vi "UI (The Advanced).vi"() -> ()   [LabVIEW 2017, in "UI.lvlib"]
doc: "The Queued Message Handler of a Worker."
uses:
  UI.lvlib
  _support/Analysis Window Type.ctl
  _support/UI State.ctl
  1af51285-6659-428e-9c15-de70f1a207c9.vi
  1756710f-d813-4077-a3f9-6f06171a4225.vi
  b1498353-a107-4479-98d0-7e76c0451ff6.vi
  242d01f8-d211-4c25-bb6c-8191a2acbe42.vi
  da0d510b-1f54-4e49-9d1f-893e7e8abfcf.vi
  e403ca69-710b-4b23-8527-f02bfa86df9b.vi
  <userlib>/_NEVSTOP/Communicable State Machine(CSM)/AdvanceAPI/CSM - Revert Arguments-Safe String.vi
  <userlib>/_NEVSTOP/Communicable State Machine(CSM)/_Shared/Trim Single-line Text.vi
  <userlib>/_NEVSTOP/Communicable State Machine(CSM)/AdvanceAPI/CSM - Make String Arguments Safe.vi
  <userlib>/_NEVSTOP/Communicable State Machine(CSM)/AdvanceAPI/CSM - Break Down Multiple States String.vi
  <userlib>/_NEVSTOP/Communicable State Machine(CSM)/AdvanceAPI/CSM - Keywords.vi
  <userlib>/_NEVSTOP/Communicable State Machine(CSM)/addons/INI-Static-Variable-Support/_Support/instances/_CSM - Read File Logger Configuration - v1.0.vi
  <userlib>/_NEVSTOP/Communicable State Machine(CSM)/addons/API-String-Arugments-Support/_Support/Convert API String Arguments to Data(variant).vi
  <userlib>/_NEVSTOP/Communicable State Machine(CSM)/addons/API-String-Arugments-Support/_Support/Query Data as API String Arguments(variant).vi
  <userlib>/_NEVSTOP/Communicable State Machine(CSM)/addons/MassData-Parameter/_support/FGV-MassData(lvlibp).vi
  <userlib>/_NEVSTOP/Communicable State Machine(CSM)/_Polymophic/Add State(s) to Queue By BOOL(Element).vi
  <userlib>/_NEVSTOP/Communicable State Machine(CSM)/_Polymophic/CSM - Replace Marks in Messages.vi
  Acquisition/Acquisition.lvlib
  Logging/Logging.lvlib
  <userlib>/_NEVSTOP/Communicable State Machine(CSM)/Communicable State Machine.lvlib
  <userlib>/_NEVSTOP/Communicable State Machine(CSM)/addons/MassData-Parameter/CSM MassData Parameter Support.lvlib
  <userlib>/_NEVSTOP/Communicable State Machine(CSM)/addons/INI-Static-Variable-Support/INI-Static-Variable-Support.lvlib
  Algorithm/Algorithm.lvlib
  <userlib>/_NEVSTOP/Communicable State Machine(CSM)/addons/Logger/CSM File Logger.lvlib
  <userlib>/_NEVSTOP/Communicable State Machine(CSM)/addons/Watchdog/CSM Watchdog.lvlib
  SoundInput-DAQ/SoundInput-DAQ.lvlib
  <userlib>/_NEVSTOP/Communicable State Machine(CSM)/_Polymophic/Build Synchronous Message with Arguments.vi
panel:
  in  "Data Source":enum16{"Simulated Waveform", "Sound Card"}(ring) caption="Data Source: \nSelect Before Running"
  out "WaveformGraph":waveform(dbl)[](graph)
  in  "Analysis Window 1":T1
  out "AnalysisWnd 1":cluster{"f0":dbl, "df":dbl, "magnitude":dbl[]}[](graph)
  in  "Analysis Window 2":T1
  out "AnalysisWnd 2":cluster{"f0":dbl, "df":dbl, "magnitude":dbl[]}[](graph)
  in  "Settings":bool
  in  "Start":bool
  in  "Stop":bool
  out "Status":string
  in  "Exit":bool
  # "Continuous Measurement and Data Logger - CSM Version"
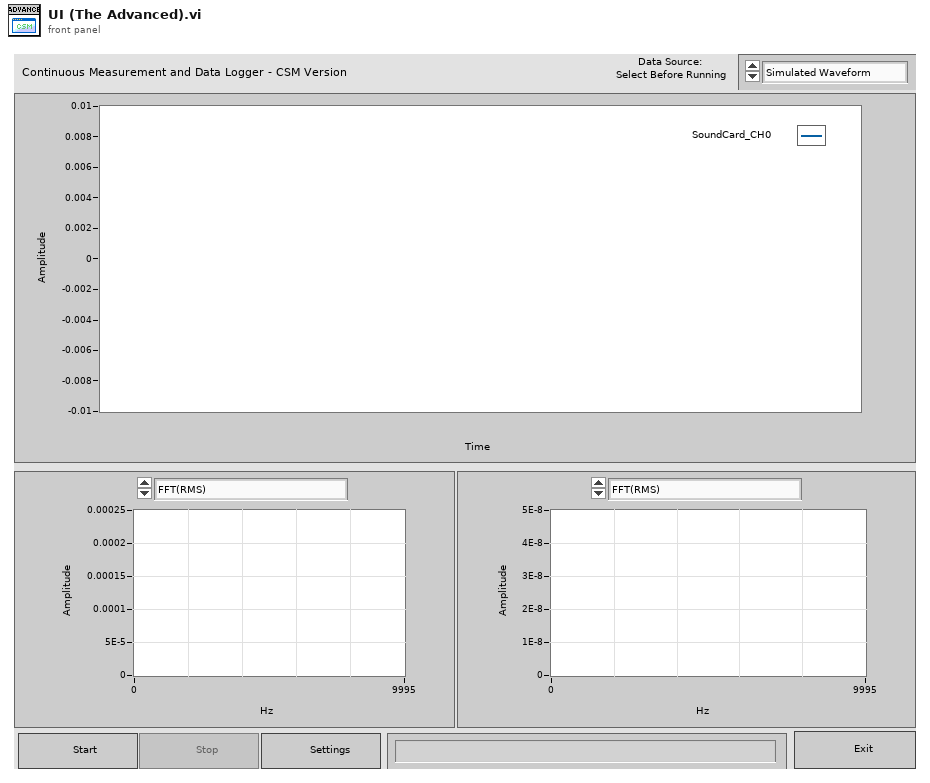
[diagram p1: front panel]
types:
  T1 = typedef "UI.lvlib/Analysis Window Type.ctl" = enum16{"FFT(RMS)", "FFT(Peak)", "Power Spectrum"}
  T2 = cluster{"Enable":bool, "Limit":cluster{"FileSize":i64, "FileNum":i32}, "Timestamp.Format":string, "AutoExit":bool}
  T3 = enum32{"Invalid", "Standard", "Closed", "Hidden", "Minimized", "Maximized"}
  T4 = enum32{"invalid app kind", "Development System", "Run Time System", "Student Edition", "Embedded LabVIEW", "Evaluation", "Custom"}
  T5 = typedef "UI.lvlib/UI State.ctl" = enum16{"Idle", "Acquiring and Logging", "Waiting for Exit", "Waiting for Exit (Acq Stopped)", "Waiting for Exit (Log Stopped)", "Waiting for Stop", "Waiting for Stop (Acq Stopped)", "Waiting for Stop (Log Stopped)"}
  T6 = enum32{"Invalid", "Default", "Floating", "Floating/Auto-Hide", "Modal"}
  T7 = typedef "Communicable State Machine.lvlib/_CSM_Response Source Message.ctl" = cluster{"‘State":string, "’Arguments":string, "’Error":errorcluster}
  T8 = cluster{"Current VI Reference":refnum<vi>, "Close Panel on Exit?":bool}
  T9 = cluster{"Core":cluster{"Current VI Reference":refnum<vi>, "Close Panel on Exit?":bool}, "UI Refs":cluster{"Start Ref":refnum<vi>, "Stop Ref":refnum<vi>, "Settings Ref":refnum<vi>, "Exit Ref":refnum<vi>, "Status Ref":refnum<vi>, "Data Ref":refnum<vi>, "Data Source Ref":refnum<vi>}, "State":T5, "Relationships":string}
  T10 = cluster{"Start Ref":refnum<vi>, "Stop Ref":refnum<vi>, "Settings Ref":refnum<vi>, "Exit Ref":refnum<vi>, "Status Ref":refnum<vi>, "Data Ref":refnum<vi>, "Data Source Ref":refnum<vi>}
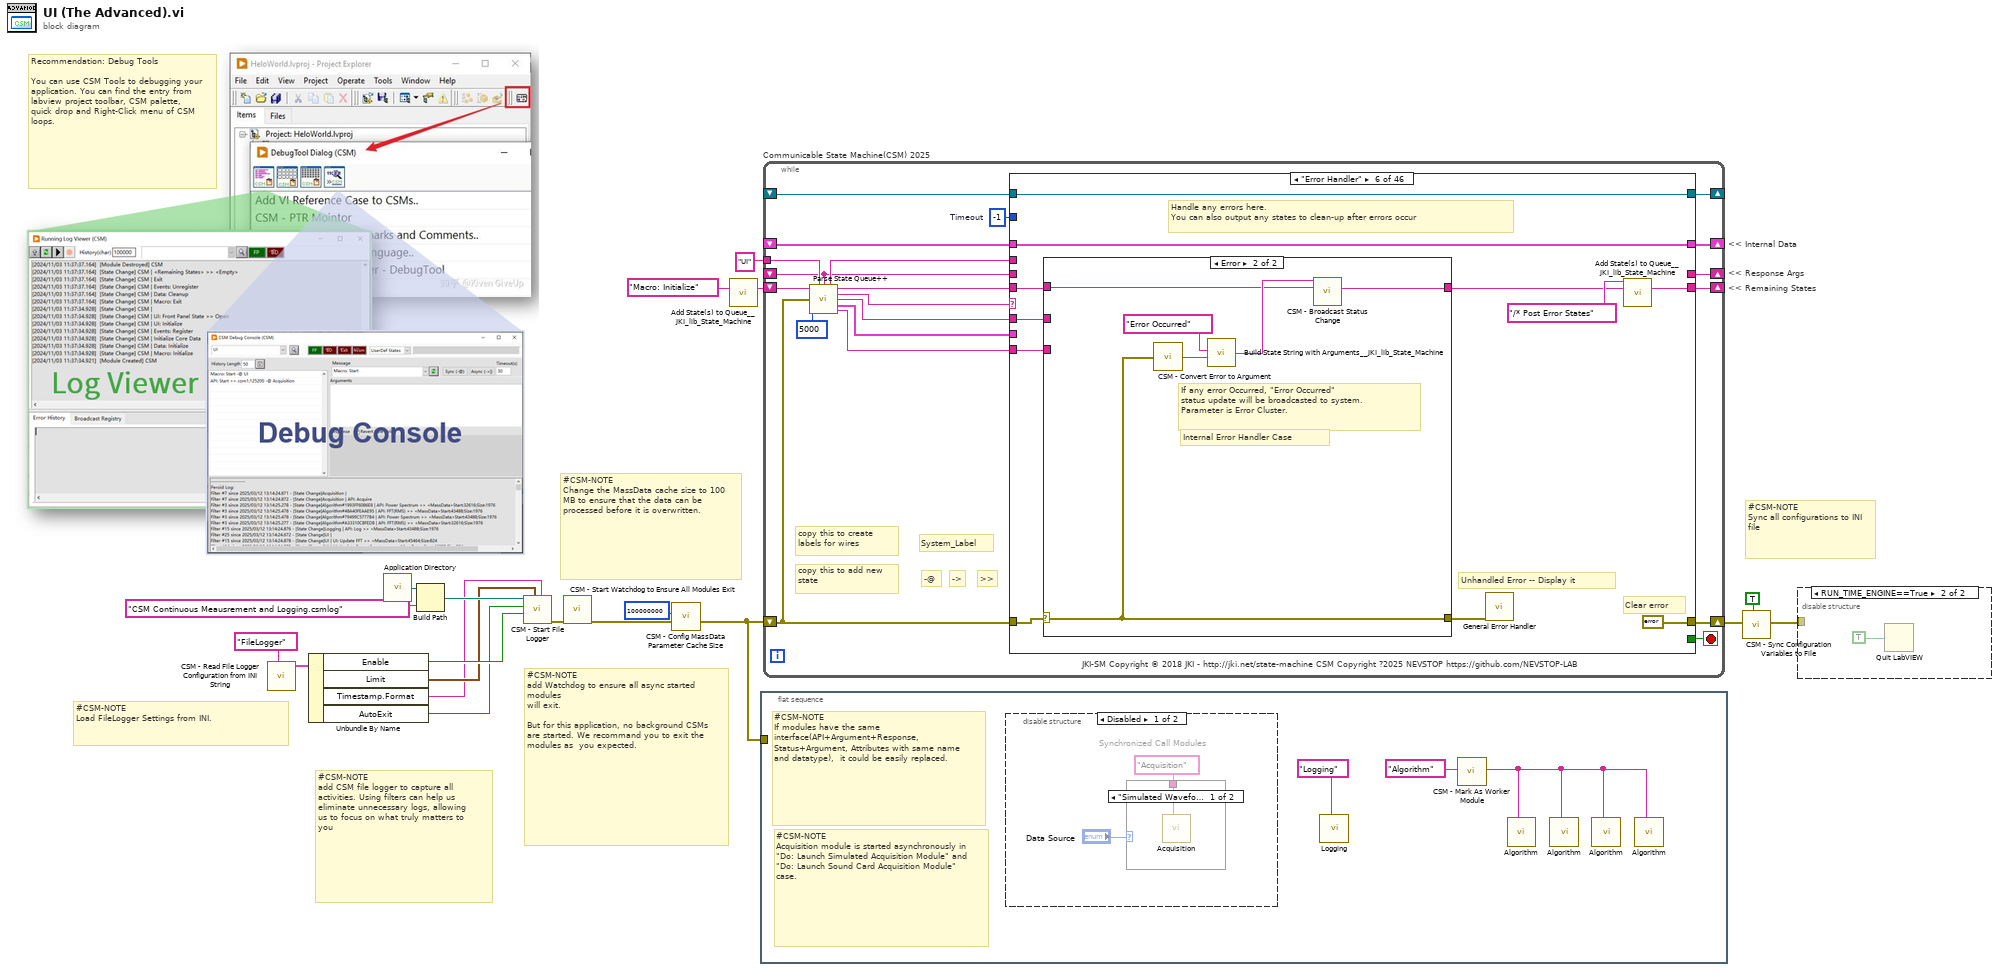
[diagram p0: block diagram]
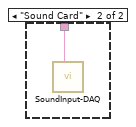
[diagram p3: hidden frame]
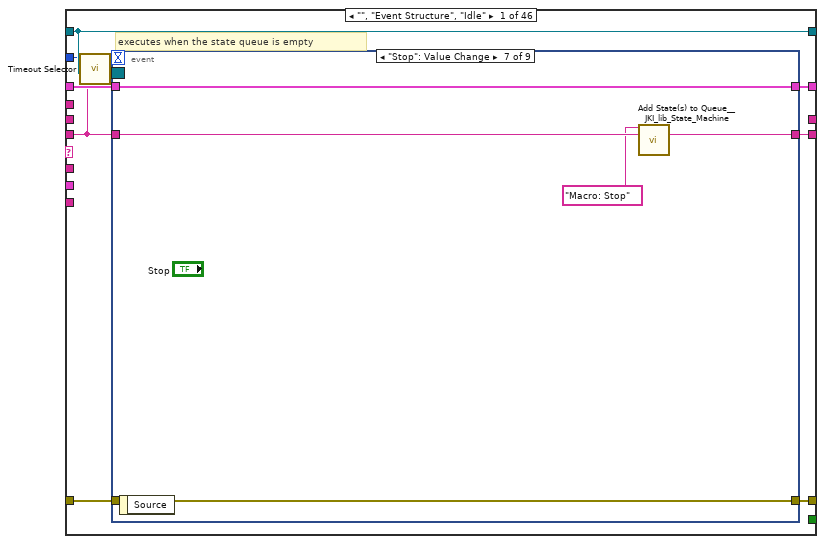
[diagram p5: hidden frame]
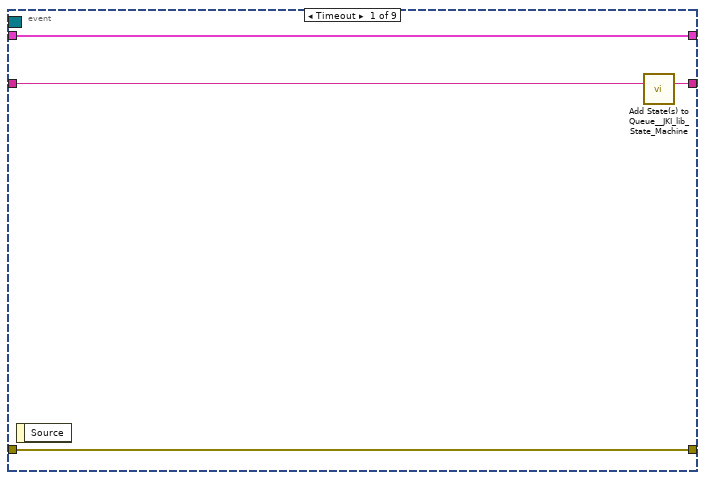
[diagram p6: hidden frame]
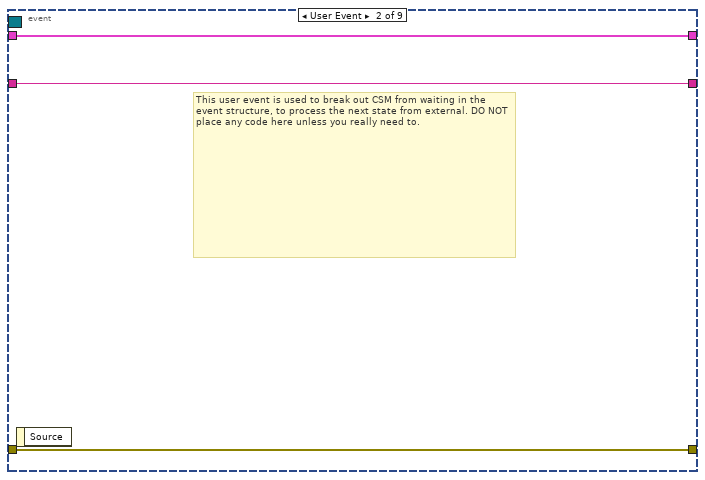
[diagram p7: hidden frame]
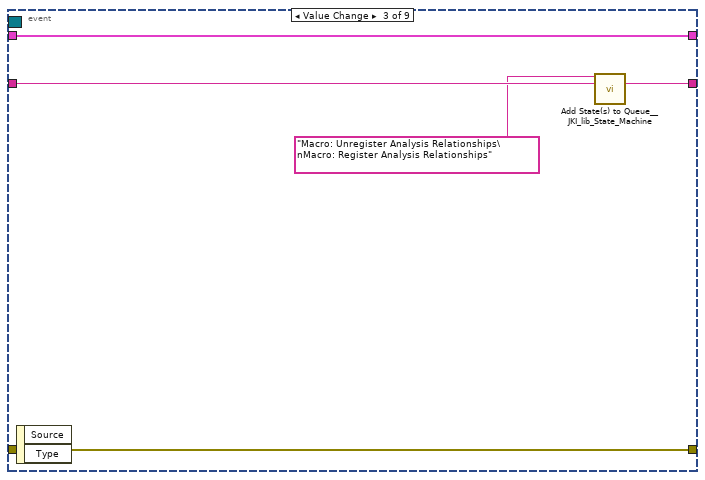
[diagram p8: hidden frame]
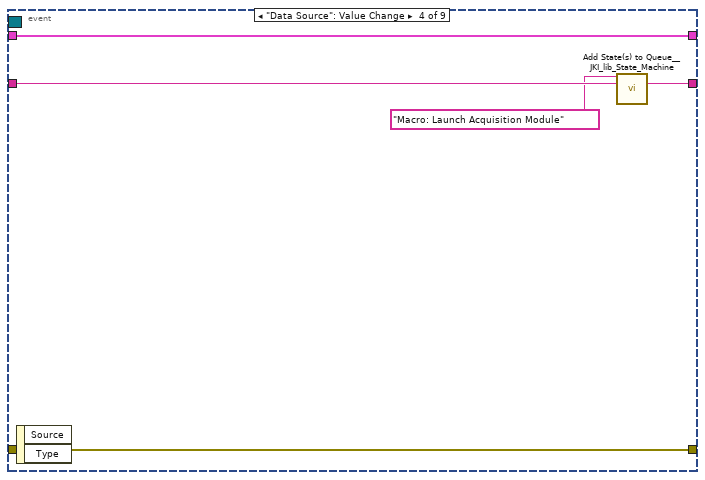
[diagram p9: hidden frame]
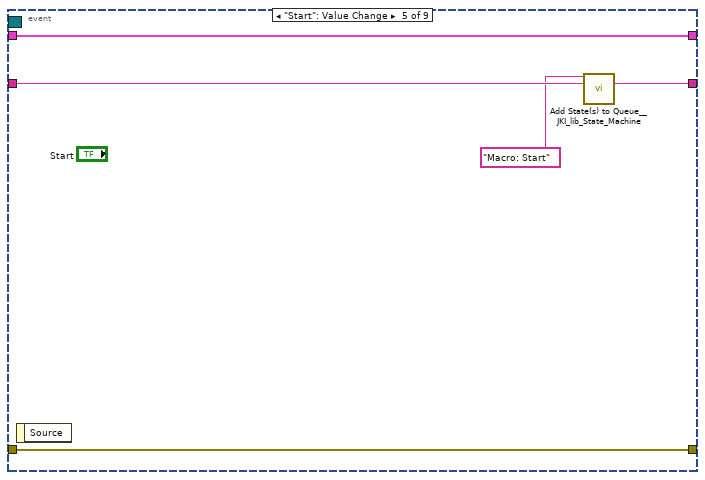
[diagram p10: hidden frame]
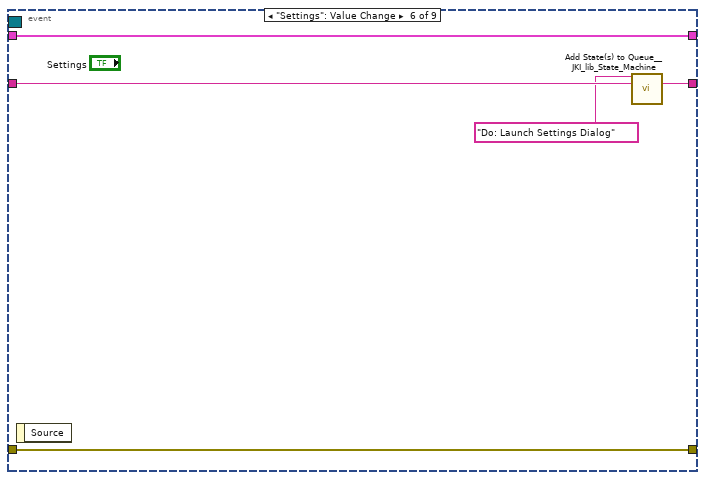
[diagram p11: hidden frame]
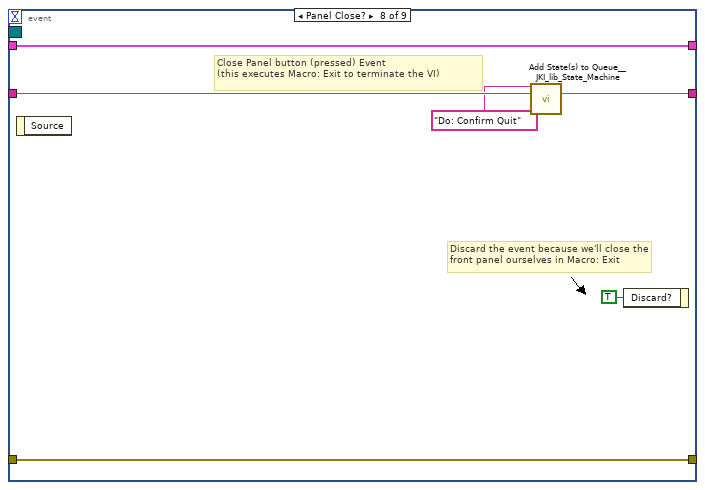
[diagram p12: hidden frame]
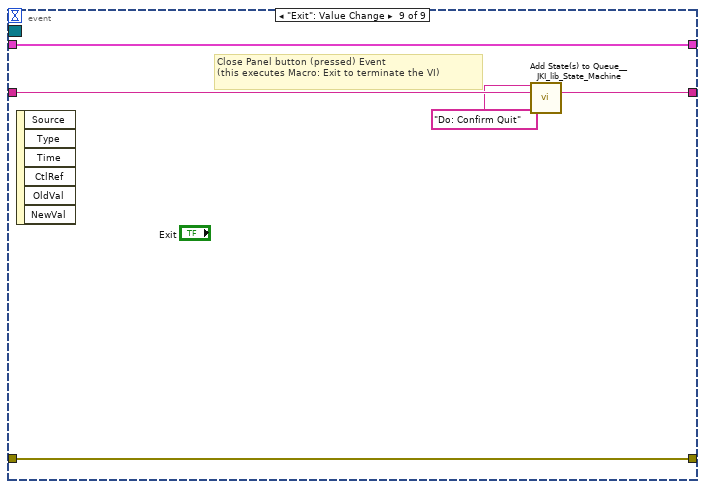
[diagram p13: hidden frame]
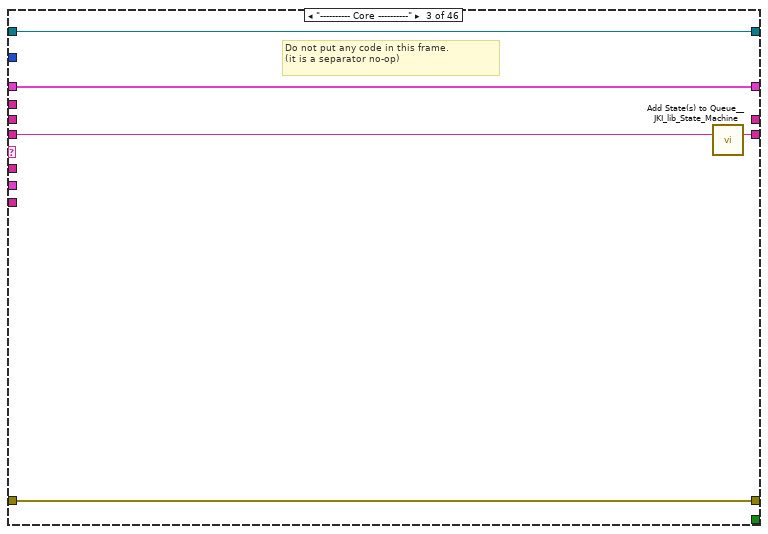
[diagram p15: hidden frame]
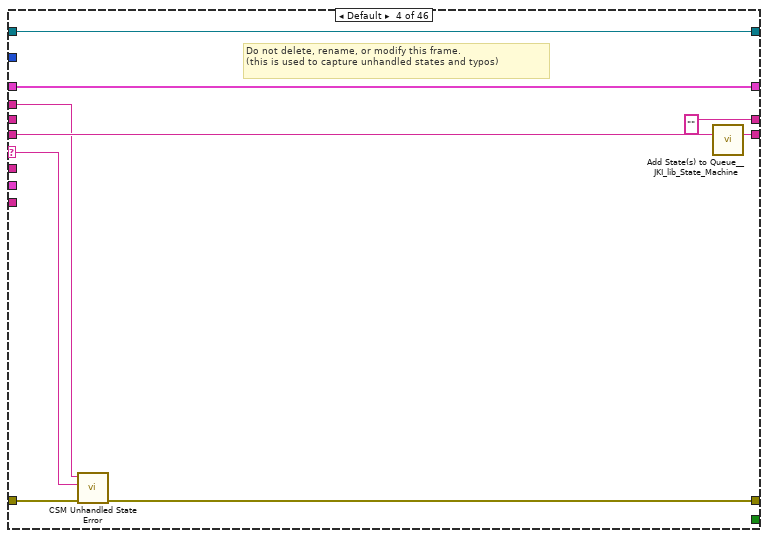
[diagram p16: hidden frame]
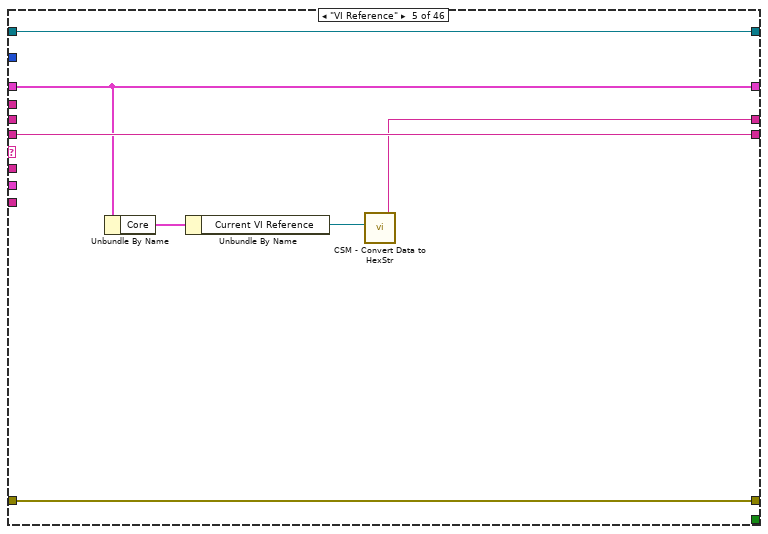
[diagram p17: hidden frame]
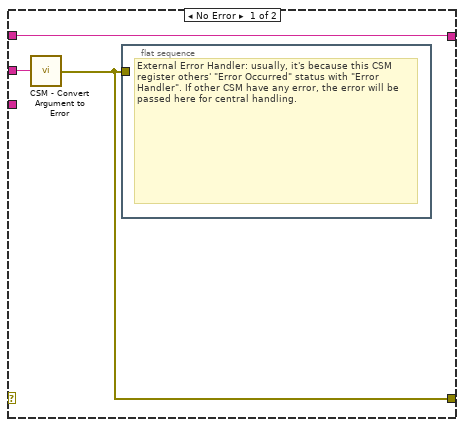
[diagram p18: hidden frame]
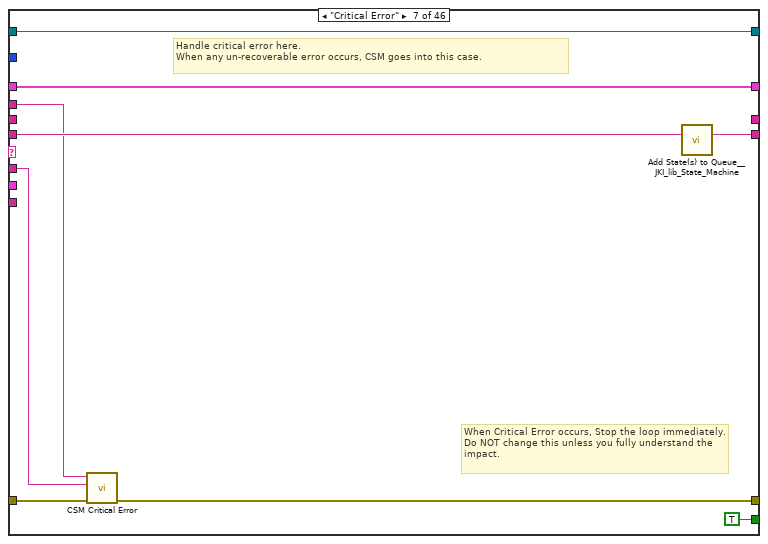
[diagram p19: hidden frame]
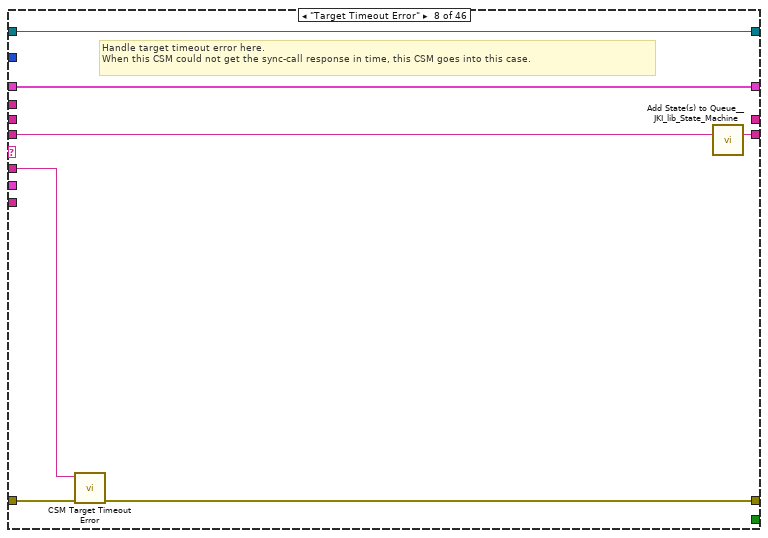
[diagram p20: hidden frame]
diagram:
  # "#CSM-NOTE\nSync all configurations to INI file"
  # "#CSM-NOTE\nChange the MassData cache size to 100 MB to ensure that the data can be processed before it is overwritten."
  # "Recommendation: Debug Tools\n\nYou can use CSM Tools to debugging your application. You can find the entry from labview project toolbar, CSM palette, quick drop and Right-Click menu of CSM loops."
  # "#CSM-NOTE\nLoad FileLogger Settings from INI."
  # "#CSM-NOTE\nadd CSM file logger to capture all activities. Using filters can help us eliminate unnecessary logs, allowing us to focus on what truly matters to you"
  # "#CSM-NOTE\nadd Watchdog to ensure all async started modules\nwill exit. \n\nBut for this application, no background CSMs are started. We recommand you to exit the modules as  you expected."
  # "<< Internal Data"
  # "<< Response Args"
  # "<< Remaining States"
  n1 = call-poly <userlib>:"CSM - Read File Logger Configuration from INI String.vi"("Section Name(\"FileLogger\")"="FileLogger" ("Section Name(\"\" as Default)")) -> ("FileLogger Configuration-v1"=w11:T2)  [unwired: 7 in, 1 out]
  n2 = Unbundle By Name(w11) -> ("Enable"=w10:bool, "Limit"=w9:cluster{"FileSize":i64, "FileNum":i32}, "Timestamp.Format"=w7:string, "AutoExit"=w8:bool)
  n3 = call <vilib>:"Application Directory.vi"() -> ("Application Directory"=w16:path)
  n4 = Build Path(base path=w16, name or relative path="CSM Continuous Meausrement and Logging.csmlog") -> (appended path=w14:path)
  n5 = call <userlib>:"CSM - Start File Logger.vi"("Timestamp Format"=w7, "Log Limit"=w9, "Watchdog? (T)"=w10, "Exit When All Module Exist? (F)"=w8, "Log File Path"=w14) -> ("error out"=w13:errorcluster)  [unwired: 4 in, 2 out]
  n6 = call <userlib>:"CSM - Start Watchdog to Ensure All Modules Exit.vi"("error in (no error)"=w13) -> ("error out"=w5:errorcluster)  [unwired: 10 in]
  n7 = call <userlib>:"CSM - Config MassData Parameter Cache Size.vi"("Error in"=w5, "Size (50M)"=100000000 ("size(1M)")) -> ("Error out"=w4:errorcluster)  [unwired: 9 in]
  n8 = call <vilib>:"Add State(s) to Queue__JKI_lib_State_Machine.vi"("State(s) in (\"\")"="Macro: Initialize") -> ("States Out"=w17:string)  [unwired: 14 in]
  n9 = flat-sequence {
    tunnel: w4 -> [_]
    frame #0 {
      # "#CSM-NOTE\nAcquisition module is started asynchronously in \"Do: Launch Simulated Acquisition Module\" and \"Do: Launch Sound Card Acquisition Module\" case."
      # "#CSM-NOTE\nIf modules have the same interface(API+Argument+Response, Status+Argument, Attributes with same name and datatype),  it could be easily replaced."
      n10 = disable-structure shown="Disabled" {
        frame Disabled {
          # "Synchronized Call Modules"
          n11 = case shown="\"Simulated Waveform\", Default" "Data Source" {
            tunnel: "Acquisition" ("Name(\"\" to use uuid)") -> [w25 w26]
            frame "Simulated Waveform", Default {
              n12 = call "Acquisition.vi"("Name(\"\" to use uuid)"=w25) -> ()  [unwired: 11 in]
            }
            frame "Sound Card" {
              n13 = call "SoundInput-DAQ.vi"("Name(\"\" to use uuid)"=w26) -> ()  [unwired: 11 in]
            }
          }
        }
        frame Enabled {
        }
      }
      n14 = call "Logging.vi"("Name(\"\" to use uuid)"="Logging" ("Name(\"\" to use uuid)")) -> ()  [unwired: 11 in]
      n15 = call <userlib>:"CSM - Mark As Worker Module.vi"("CSM Name"="Algorithm" ("Name(\"\" to use uuid)")) -> ("CSM Name (Marked As Worker)"=w20:string)  [unwired: 9 in]
      n16 = call "Algorithm.vi"("Name(\"\" to use uuid)"=w20) -> ()  [unwired: 11 in]
      n17 = call "Algorithm.vi"("Name(\"\" to use uuid)"=w20) -> ()  [unwired: 11 in]
      n18 = call "Algorithm.vi"("Name(\"\" to use uuid)"=w20) -> ()  [unwired: 11 in]
      n19 = call "Algorithm.vi"("Name(\"\" to use uuid)"=w20) -> ()  [unwired: 11 in]
    }
  }
  n20 = while "Communicable State Machine(CSM) 2025" {
    shift-right: [w41] -> _
    shift-left: _ -> [w40]
    shift-right: [w44] -> w2
    shift-left: w4 -> [w38]
    shift-right: [w43] -> _
    shift-left: w17 -> [w45]
    tunnel: "UI" ("Name(\"\" to use uuid)") -> [w33]
    shift-right: [w36] -> _
    shift-left: _ -> [w28]
    shift-right: [w35] -> _
    shift-left: _ -> [w34]
    stop <- w42 stop-if-true
    w39 = -1  # Timeout
    # "JKI-SM Copyright © 2018 JKI - http://jki.net/state-machine CSM Copyright ?2025 NEVSTOP https://github.com/NEVSTOP-LAB"
    # "copy this to add new state"
    # ">>"
    # "->"
    # "-@"
    # "copy this to create labels for wires"
    # "System_Label"
    n21 = call <userlib>:"Parse State Queue++.vi"("State Queue"=w45, "Name (\"\" to Use UUID)"=w33, "Response Arguments"=w28, "Previous Error"=w38, "Response Timeout (-2 Use Global Settings)"=5000 ("Response Timeout(1000ms)")) -> ("Name Used"=w29:string, "Remaining States"=w46:string, "Current State"=w32:string, "Arguments"=w27:string, "Additional Information"=w31:T7, "Source CSM"=w30:string)  [unwired: 5 in]
    n22 = case shown="\"Error Handler\"" w32 {
      selector: w32 -> [_ _ _ w109 _ _ _ _ _ _ _ _ _ _ _ _ _ _ _ _ _ _ _ _ _ _ _ _ _ _ _ _ _ _ _ _ _ _ _ _ _ _ _ _ _ _]
      tunnel: w46 -> [w47 w101 w107 w116 w122 w127 w150 w158 w165 w169 w173 w188 w195 w200 w209 w215 w222 w229 w234 w240 w244 w250 w271 w283 w296 w304 w320 w394 w403 w416 w423 w428 w435 w440 w454 w462 w473 w484 w502 w527 w533 w541 w579 w604 w625 w640]
      tunnel: w27 -> [_ _ _ _ _ w125 w145 w154 w161 _ _ _ _ _ _ w213 w219 _ _ _ _ _ _ _ _ w299 w314 w389 w407 w413 w420 _ _ _ _ _ _ _ _ _ w528 _ _ _ _ _]
      tunnel: w40 -> [w54 w100 w104 w114 w121 w133 w151 w156 w163 w168 w172 w181 w193 w197 _ w212 w220 w224 w231 w239 w243 w247 w257 w273 w286 w302 w316 w392 w409 w415 w422 w425 w432 w443 w457 w469 w476 w480 w500 w524 w530 w534 w574 w603 w624 w639]
      tunnel: [w53 w102 w105 w111 w123 errorcluster {"status"=FALSE, "code"=0, "source"=""} ("error out") w146 w153 w160 w170 w174 w185 w192 w198 w203 w211 w218 w225 w232 w235 w242 w248 w269 w284 w297 w300 w317 w386 w405 w412 w419 w426 w433 w444 w458 w471 w479 w488 _ w525 w531 w535 _ w596 w612 w627] -> w44
      tunnel: w38 -> [w52 w102 w105 w108 w123 w131 w152 w159 w166 w170 w174 w185 w192 w198 w203 _ _ w226 w232 _ w245 w248 w269 w284 w297 w301 w318 _ _ _ _ w426 w433 w444 w458 w471 w479 w488 _ w525 w531 _ _ _ _ _]
      tunnel: [w55 w101 w106 w115 w122 w129 w149 w157 w164 w169 w173 w187 w194 w199 w208 w215 w222 w228 w233 w240 w244 w249 w270 w283 w296 w303 w319 w394 w404 w416 w423 w427 w434 w441 w455 w463 w474 w485 w501 w526 w532 w541 w572 w604 w625 w640] -> w43
      tunnel: [_ _ _ _ _ _ TRUE _ _ _ _ _ TRUE _ _ _ _ _ _ _ _ _ _ _ _ _ _ _ _ _ _ _ _ _ _ _ _ _ _ _ _ _ _ _ _ _] -> w42
      tunnel: [w51 w100 w104 w114 w121 w133 w151 w156 w163 w168 w172 w186 w193 w197 w202 w210 w216 w224 w231 w239 w243 w247 w256 w273 w286 w302 w316 w392 w409 w415 w422 w425 w432 w443 w453 w460 w475 w486 w500 w524 w530 w534 w573 w603 w624 w639] -> w41
      tunnel: w39 -> [w49 _ _ _ _ _ _ _ _ _ _ _ _ _ _ _ _ _ _ _ _ _ _ _ _ _ _ _ _ _ _ _ _ _ _ _ _ _ _ _ _ _ _ _ _ _]
      tunnel: w30 -> [_ _ _ _ _ w124 _ _ _ _ _ _ _ _ _ _ _ _ _ _ _ _ _ _ _ _ _ _ _ _ _ _ _ _ _ _ _ _ _ _ _ _ _ _ _ _]
      tunnel: w31 -> [_ _ _ _ _ _ _ _ _ _ _ _ _ _ _ _ _ _ _ _ _ _ _ _ _ _ _ _ _ _ _ _ _ _ _ _ _ _ _ _ _ _ _ _ _ _]
      tunnel: [_ _ _ "" w117 _ _ _ _ _ _ _ _ _ _ _ w217 _ _ _ _ _ _ _ _ _ _ _ _ _ _ _ _ _ _ _ _ _ _ _ _ _ _ _ _ _] -> w36
      tunnel: [w50 w99 w103 w112 w120 w132 w147 w155 w162 w167 w171 w175 w190 w196 w206 w214 w221 w223 w230 w238 w241 w246 w268 w282 w295 w298 w313 w393 w408 w414 w421 w424 w431 w442 w456 w470 w478 w487 w493 w523 w529 w542 w578 w602 w623 w638] -> w35
      tunnel: w34 -> [w50 w99 w103 w112 w120 w132 w147 w155 w162 w167 w171 w175 w190 w196 w206 w214 w221 w223 w230 _ w241 w246 w268 w282 w295 w298 w313 w393 w408 w414 w421 w424 w431 w442 w456 w470 w478 w487 w493 w523 w529 w542 w578 w602 w623 w638]
      tunnel: w29 -> [_ _ _ w110 _ _ w144 _ _ _ _ _ _ _ _ _ _ _ _ w237 _ _ _ _ _ _ _ _ _ _ _ _ _ _ _ _ _ _ w491 _ _ w537 _ w599 _ _]
      tunnel: w28 -> [_ _ _ _ _ _ _ _ _ _ _ _ _ _ _ _ _ _ _ _ _ _ _ _ _ _ _ _ _ _ _ _ _ _ _ _ _ _ _ _ _ _ _ _ _ _]
      frame "", "Event Structure", "Idle" {
        # "executes when the state queue is empty"
        n23 = call <userlib>:"Timeout Selector.vi"("Remaining States"=w47, "Timeout Expected"=w49) -> ("Timeout"=w48:i32)  [unwired: 5 in]
        n24 = event shown="[6] \"Stop\": Value Change" {
          selector: w50 -> [_ _ _ _ _ _ _ _ _]
          dyn-events: _ -> [_ _ _ _ _ _ _ _ _]
          timeout: w48 -> [_ _ _ _ _ _ _ _ _]
          tunnel: w47 -> [w59 w61 w64 w69 w74 w79 w84 w93 w98]
          tunnel: [w58 w61 w65 w70 w75 w80 w85 w92 w97] -> w55
          tunnel: w54 -> [w56 w62 w66 w71 w76 w81 w86 w90 w95]
          tunnel: [w57 w60 w67 w72 w77 w82 w87 w91 w96] -> w53
          tunnel: w52 -> [w57 w60 w67 w72 w77 w82 w87 w91 w96]
          tunnel: [w56 w62 w66 w71 w76 w81 w86 w90 w95] -> w51
          event Timeout {
            n25 = event-data() -> ()  [unwired: 1 in, 1 out]
            n26 = call <vilib>:"Add State(s) to Queue__JKI_lib_State_Machine.vi"("State(s) in (\"\")"=w59) -> ("States Out"=w58:string)  [unwired: 14 in]
          }
          event User Event {
            # "This user event is used to break out CSM from waiting in the event structure, to process the next state from external. DO NOT place any code here unless you really need to."
            n27 = event-data() -> ()  [unwired: 1 in, 1 out]
          }
          event Value Change {
            n28 = event-data() -> ()  [unwired: 1 in, 2 out]
            n29 = call <vilib>:"Add State(s) to Queue__JKI_lib_State_Machine.vi"("State(s) in Front (\"\")"="Macro: Unregister Analysis Relationships\nMacro: Register Analysis Relationships" ("State(s) in Front (\"\")"), "State(s) in (\"\")"=w64) -> ("States Out"=w65:string)  [unwired: 13 in]
          }
          event "Data Source": Value Change {
            n30 = event-data() -> ()  [unwired: 1 in, 2 out]
            n31 = call <vilib>:"Add State(s) to Queue__JKI_lib_State_Machine.vi"("State(s) in Front (\"\")"="Macro: Launch Acquisition Module" ("State(s) in Front (\"\")"), "State(s) in (\"\")"=w69) -> ("States Out"=w70:string)  [unwired: 13 in]
          }
          event "Start": Value Change {
            n32 = event-data() -> ()  [unwired: 1 in, 1 out]
            n33 = call <vilib>:"Add State(s) to Queue__JKI_lib_State_Machine.vi"("State(s) in Front (\"\")"="Macro: Start" ("State(s) in Front (\"\")"), "State(s) in (\"\")"=w74) -> ("States Out"=w75:string)  [unwired: 13 in]
          }
          event "Settings": Value Change {
            n34 = event-data() -> ()  [unwired: 1 in, 1 out]
            n35 = call <vilib>:"Add State(s) to Queue__JKI_lib_State_Machine.vi"("State(s) in Front (\"\")"="Do: Launch Settings Dialog" ("State(s) in Front (\"\")"), "State(s) in (\"\")"=w79) -> ("States Out"=w80:string)  [unwired: 13 in]
          }
          event "Stop": Value Change {
            n36 = event-data() -> ()  [unwired: 1 in, 1 out]
            n37 = call <vilib>:"Add State(s) to Queue__JKI_lib_State_Machine.vi"("State(s) in Front (\"\")"="Macro: Stop" ("State(s) in Front (\"\")"), "State(s) in (\"\")"=w84) -> ("States Out"=w85:string)  [unwired: 13 in]
          }
          event Panel Close? {
            # "Discard the event because we'll close the front panel ourselves in Macro: Exit"
            # "Close Panel button (pressed) Event\n(this executes Macro: Exit to terminate the VI)"
            n38 = event-data() -> ()  [unwired: 1 in, 1 out]
            n39 = call <vilib>:"Add State(s) to Queue__JKI_lib_State_Machine.vi"("State(s) in Front (\"\")"="Do: Confirm Quit", "State(s) in (\"\")"=w93) -> ("States Out"=w92:string)  [unwired: 13 in]
            n40 = event-data("Discard?"=TRUE) -> ()  [unwired: 1 in, 1 out]
          }
          event "Exit": Value Change {
            # "Close Panel button (pressed) Event\n(this executes Macro: Exit to terminate the VI)"
            n41 = event-data() -> ()  [unwired: 1 in, 6 out]
            n42 = call <vilib>:"Add State(s) to Queue__JKI_lib_State_Machine.vi"("State(s) in Front (\"\")"="Do: Confirm Quit", "State(s) in (\"\")"=w98) -> ("States Out"=w97:string)  [unwired: 13 in]
          }
        }
      }
      frame "CSM Documentation" {
        # "CSM Documentation"
        # "State Syntax:\nStateCategory: State >> Argument -@ CSMName\nStateCategory: State >> Argument -> CSMName\n\nLine Terminator: Line feed"
        # "Commenting:\nTo add a comment use \"//\" or \"#\" and all text to the right will be ignored\nCommenting Example:\nUI: Initialize // This initializes the UI\n// Another comment line"
        # "Example:\nUI: Help >> About -@Main\nUI: Help >> About ->Main\n\nWhere \"UI\" is the state category\nWhere \"Help\" is the state\nWhere \"About\" is the argument\nWhere \"Main\" is the Name of CSM,which actually run the \"UI: Help >> About\"\n\n    \"-@\" stands for sync state. Current CSM will wait until the state is finished. \n            - if \"Main\" named CSM does not exist, \"Target Error\" will occur.\n            - if \"Main\" named CSM is in another sync remote state, \"Target Busy Error\" will occur.\n            - if \"Main\" named CSM could not finish the state in time, \"Target Timeout Error\" will occur.\n            - if everything is right. \"Response\" will occur with Argument back from \"Main\" named CSM. \n\n    \"->\" stands for async state. Current CSM will post the state and continue to next state in next iteration.\n            - if \"Main\" named CSM does not exist, \"Target Error\" will occur.\n            - if everything is right. \"Async Message Posted\" will occur.\n            - After State is finished. Caller will receive a \"Async Response\" state from callee.\n\nWhen duplicated name is used for multiple CSM module or some framework problem happens, \"Critical Error\" will occur."
      }
      frame "---------- Core ----------" {
        # "Do not put any code in this frame.\n(it is a separator no-op)"
        n43 = call <vilib>:"Add State(s) to Queue__JKI_lib_State_Machine.vi"("State(s) in (\"\")"=w107) -> ("States Out"=w106:string)  [unwired: 14 in]
      }
      frame Default {
        # "Do not delete, rename, or modify this frame.\n(this is used to capture unhandled states and typos)"
        n44 = call <userlib>:"CSM Unhandled State Error.vi"("error in (no error)"=w108, "Undefined State"=w109, "CSM Name"=w110) -> ("error out"=w111:errorcluster)  [unwired: 8 in]
        n45 = call <vilib>:"Add State(s) to Queue__JKI_lib_State_Machine.vi"("State(s) in (\"\")"=w116) -> ("States Out"=w115:string)  [unwired: 14 in]
      }
      frame "VI Reference" {
        n46 = Unbundle By Name(w121) -> ("Core"=w119:T8)
        n47 = Unbundle By Name(w119) -> ("Current VI Reference"=w118:refnum<vi>)
        n48 = call <userlib>:"CSM - Convert Data to HexStr.vi"("Variant"=w118) -> ("HEX String (0-9,A-F)"=w117:string)  [unwired: 8 in]
      }
      frame "Error Handler" {
        # "Unhandled Error -- Display it"
        # "Handle any errors here.\nYou can also output any states to clean-up after errors occur"
        # "Clear error"
        n49 = case shown="Error" w131 {
          selector: w131 -> [_ w138]
          tunnel: [w136 w140] -> w128
          tunnel: w127 -> [w136 w139]
          tunnel: [w135 w138] -> w126
          tunnel: w125 -> [w137 _]
          tunnel: w124 -> [_ _]
          frame No Error {
            n50 = call <userlib>:"CSM - Convert Argument to Error.vi"("Argument"=w137) -> ("Error"=w135:errorcluster)  [unwired: 4 in]
            n51 = flat-sequence {
              tunnel: w135 -> [_]
              frame #0 {
                # "External Error Handler: usually, it's because this CSM register others' \"Error Occurred\" status with \"Error Handler\". If other CSM have any error, the error will be passed here for central handling."
              }
            }
          }
          frame Error {
            # "Internal Error Handler Case"
            # "If any error Occurred, \"Error Occurred\" \nstatus update will be broadcasted to system.\nParameter is Error Cluster."
            n52 = call <userlib>:"CSM - Convert Error to Argument.vi"("Error"=w138) -> ("Argument"=w142:string)  [unwired: 4 in]
            n53 = call <vilib>:"Build State String with Arguments__JKI_lib_State_Machine.vi"("Arguments (\"\")"=w142, "State"="Error Occurred" ("Status with Arguments")) -> ("State with Arguments"=w141:string)  [unwired: 4 in]
            n54 = call <userlib>:"CSM - Broadcast Status Change.vi"("Status With Arguments"=w141, "State Queue"=w139) -> ("Remaining States"=w140:string)  [unwired: 13 in]
          }
        }
        n55 = call <vilib>:"General Error Handler.vi"("error in (no error)"=w126) -> ()  [unwired: 10 in, 5 out]
        n56 = call <vilib>:"Add State(s) to Queue__JKI_lib_State_Machine.vi"("State(s) in Front (\"\")"="/* Post Error States", "State(s) in (\"\")"=w128) -> ("States Out"=w129:string)  [unwired: 13 in]
      }
      frame "Critical Error" {
        # "Handle critical error here.\nWhen any un-recoverable error occurs, CSM goes into this case."
        # "When Critical Error occurs, Stop the loop immediately. Do NOT change this unless you fully understand the impact."
        n57 = call <userlib>:"CSM Critical Error.vi"("error in (no error)"=w152, "Arugments (As Reason)"=w145, "CSM Name"=w144) -> ("error out"=w146:errorcluster)  [unwired: 8 in]
        n58 = call <vilib>:"Add State(s) to Queue__JKI_lib_State_Machine.vi"("State(s) in (\"\")"=w150) -> ("States Out"=w149:string)  [unwired: 14 in]
      }
      frame "Target Timeout Error" {
        # "Handle target timeout error here.\nWhen this CSM could not get the sync-call response in time, this CSM goes into this case."
        n59 = call <userlib>:"CSM Target Timeout Error.vi"("error in (no error)"=w159, "Arguments (As CSM Name)"=w154) -> ("error out"=w153:errorcluster)  [unwired: 9 in]
        n60 = call <vilib>:"Add State(s) to Queue__JKI_lib_State_Machine.vi"("State(s) in (\"\")"=w158) -> ("States Out"=w157:string)  [unwired: 14 in]
      }
      frame "Target Error" {
        # "Handle target error here.\nWhen this CSM try to communicate with an un-existed CSM, this CSM goes into this case."
        n61 = call <userlib>:"CSM Target Error.vi"("error in (no error)"=w166, "Arguments (As CSM Name)"=w161) -> ("error out"=w160:errorcluster)  [unwired: 9 in]
        n62 = call <vilib>:"Add State(s) to Queue__JKI_lib_State_Machine.vi"("State(s) in (\"\")"=w165) -> ("States Out"=w164:string)  [unwired: 14 in]
      }
      frame "Async Response", "Response" {
        # "Handle Async-call Response (\"Async Response\" for ->)"
        # "Handle Sync-call Response (\"Response\" for -@)"
        # "After Message is executed, CSM+ goes to this state for receive the response. \n    For Async Message(->), \"Async Response\" is used. This CSM will goes to \"Async Message Posted\" immediately and receive the \"Async Response\" after the callee finishes the message.\n    For Sync Message(@),  This CSM will wait until the message is done and immediately goes to \"Response\""
      }
      frame "Async Message Posted" {
        # "Handle post action for async message (->)."
        # "After Async Message is posted (->), CSM+ goes to this state for post-action. You can use Argument - State to tell which Async Message is called."
      }
      frame "Initialize Core Data" {
        # "Do not delete, rename, or modify this frame.\n(this is used to determine panel behavior on exit)"
        # "originally closed?"
        # "exe?"
        # "If panel starts closed or is an EXE, then close it when we exit"
        n63 = property class="VI"() -> ("FP.State"=w178:T3)  [unwired: 2 in, 2 out]
        n64 = property class="App"() -> ("App.Kind"=w184:T4)  [unwired: 2 in, 2 out]
        n65 = control-ref of="Current VI Reference"() -> (w179:refnum<vi>)
        n66 = Equal?(x=w178, y=T3."Closed" ("Front Panel Window:State")) -> (x = y?=w176:bool)
        n67 = Equal?(x=w184, y=T4."Run Time System" ("Application:Kind")) -> (x = y?=w182:bool)
        n68 = Or(x=w176, y=w182) -> (x .or. y?=w180:bool)
        n69 = Bundle By Name(cluster=w181, "Core.Current VI Reference"=w179, "Core.Close Panel on Exit?"=w180) -> (w186:T9)
        n70 = call <vilib>:"Add State(s) to Queue__JKI_lib_State_Machine.vi"("State(s) in (\"\")"=w188) -> ("States Out"=w187:string)  [unwired: 14 in]
      }
      frame "Exit" {
        # "Do not put any code in this frame.\n(No errors that occur here will be handled.)"
        n71 = local write "Status"("Exit" ("Exit String")) -> ()
        n72 = call <vilib>:"Add State(s) to Queue__JKI_lib_State_Machine.vi"("State(s) in (\"\")"=w195) -> ("States Out"=w194:string)  [unwired: 14 in]
      }
      frame "---------- Data ----------" {
        # "Do not put any code in this frame.\n(It is a separator no-op. You can make a copy of this frame to create a new Data frame)"
        n73 = call <vilib>:"Add State(s) to Queue__JKI_lib_State_Machine.vi"("State(s) in (\"\")"=w200) -> ("States Out"=w199:string)  [unwired: 14 in]
      }
      frame "Data: Initialize" {
        w201 = ""  # Relationships
        w204 = UI_State."Idle"  # State
        w205 = T10 {"Start Ref"=refnum, "Stop Ref"=refnum, "Settings Ref"=refnum, "Exit Ref"=refnum, "Status Ref"=refnum, "Data Ref"=refnum, "Data Source Ref"=refnum}  # UI Refs
        w207 = T8 {"Current VI Reference"=refnum, "Close Panel on Exit?"=FALSE}  # Core
        # "Initialize the shift-register data, here.\n(data names are defined by what you wire into the bundle function)"
        n74 = Bundle("Core"=w207, "UI Refs"=w205, "State"=w204, "Relationships"=w201) -> (w202:T9)  [unwired: 1 in]
        n75 = call <vilib>:"Add State(s) to Queue__JKI_lib_State_Machine.vi"("State(s) in (\"\")"=w209) -> ("States Out"=w208:string)  [unwired: 14 in]
      }
      frame "Data: Set Configuration" {
        n76 = call "Convert API String Arguments to Data.vim"("Reference Type"=w212, "API String"=w213) -> ("error out"=w211:errorcluster, "Data"=w210:T9)  [unwired: 6 in]
      }
      frame "Data: Get Configuration", "Data: Get Internal Data" {
        n77 = call "Query Data as API String Arguments.vim"("Name"=w219, "Cluster Data"=w220) -> ("error"=w218:errorcluster, "API String"=w217:string, "Cluster Data (dup)"=w216:T9)  [unwired: 7 in]
      }
      frame "Data: Cleanup" {
        # "Cleanup any data and references, here.\n(this is called automatically, by the Macro: Exit)"
        n78 = Unbundle By Name(w224) -> ("Core.Current VI Reference"=w227:refnum<vi>)
        n79 = Close Reference(reference=w227, error in (no error)=w226) -> (error out=w225:errorcluster)
        n80 = call <vilib>:"Add State(s) to Queue__JKI_lib_State_Machine.vi"("State(s) in (\"\")"=w229) -> ("States Out"=w228:string)  [unwired: 14 in]
      }
      frame "---------- Events ----------" {
        # "Do not put any code in this frame.\n(It is a separator no-op. You can make a copy of this frame to create a new UI frame)"
        n81 = call <vilib>:"Add State(s) to Queue__JKI_lib_State_Machine.vi"("State(s) in (\"\")"=w234) -> ("States Out"=w233:string)  [unwired: 14 in]
      }
      frame "Events: Register" {
        # "Register message event to break Waiting in Event structure."
        n82 = call <userlib>:"CSM - Get New State Notifier Event.vi"("Name (\"\" to Use UUID)"=w237) -> ("error out"=w235:errorcluster, "New State Notifier Event"=w236:refnum<user-event>)  [unwired: 9 in]
        n83 = register-events(w236) -> (reference out=w238:refnum<event-registration>)  [unwired: 2 in, 1 out]
      }
      frame "Events: Unregister" {
        n84 = Unregister For Events(event registration refnum=w241, error in=w245) -> (error out=w242:errorcluster)
      }
      frame "---------- UI ----------" {
        # "Do not put any code in this frame.\n(It is a separator no-op. You can make a copy of this frame to create a new UI frame)"
        n85 = call <vilib>:"Add State(s) to Queue__JKI_lib_State_Machine.vi"("State(s) in (\"\")"=w250) -> ("States Out"=w249:string)  [unwired: 14 in]
      }
      frame "UI: Initialize" {
        w254 = cluster{"f0":dbl, "df":dbl, "magnitude":dbl[]}[] [] ("FFT")
        # "Initialize the User Interface, here.\n(this is called automatically, by the Macro: Init)"
        n86 = control-ref of="WaveformGraph"() -> (w260:refnum<vi>)
        n87 = control-ref of="Start"() -> (w265:refnum<vi>)
        n88 = control-ref of="Stop"() -> (w264:refnum<vi>)
        n89 = control-ref of="Settings"() -> (w266:refnum<vi>)
        n90 = control-ref of="Exit"() -> (w267:refnum<vi>)
        n91 = control-ref of="Status"() -> (w261:refnum<vi>)
        n92 = control-ref of="Data Source"() -> (w251:refnum<vi>)
        n93 = local write "AnalysisWnd 2"(w254) -> ()
        n94 = property on="AnalysisWnd 1" class="WFGraph (strict)"("Value"=w254) -> ()  [unwired: 2 in, 2 out]
        n95 = Bundle By Name(cluster=w257, "UI Refs.Start Ref"=w265, "UI Refs.Stop Ref"=w264, "UI Refs.Settings Ref"=w266, "UI Refs.Exit Ref"=w267, "UI Refs.Status Ref"=w261, "UI Refs.Data Ref"=w260, "UI Refs.Data Source Ref"=w251) -> (w256:T9)
        n96 = Build Array(w265, w267, w266, w251) -> (w263:refnum<vi>[])
        n97 = Build Array(w264) -> (w262:refnum<vi>[])
        n98 = property on="WaveformGraph" class="WFChart (strict)"("History Data"=waveform(dbl)[][] []) -> ()  [unwired: 2 in, 2 out]
        n99 = call "Set Enable State on Multiple Controls.vi"("Enable?"=TRUE, "Controls"=w263) -> ()  [unwired: 10 in]
        n100 = call "Set Enable State on Multiple Controls.vi"("Enable?"=FALSE, "Controls"=w262) -> ()  [unwired: 10 in]
        n101 = local write "Analysis Window 1"(Analysis_Window_Type."FFT(RMS)" ("Analysis Window 1")) -> ()
        n102 = local write "Analysis Window 2"(Analysis_Window_Type."Power Spectrum" ("Analysis Window 2")) -> ()
        n103 = call <vilib>:"Add State(s) to Queue__JKI_lib_State_Machine.vi"("State(s) in (\"\")"=w271) -> ("States Out"=w270:string)  [unwired: 14 in]
      }
      frame "UI: Update When Start" {
        # "Enable: Stop\nDisable: Start, Exit, Settings"
        n104 = Unbundle By Name(w273) -> ("UI Refs.Stop Ref"=w279:refnum<vi>, "UI Refs.Start Ref"=w278:refnum<vi>, "UI Refs.Exit Ref"=w277:refnum<vi>, "UI Refs.Settings Ref"=w276:refnum<vi>, "UI Refs.Data Source Ref"=w272:refnum<vi>)
        n105 = Build Array(w278, w277, w276, w272) -> (w281:refnum<vi>[])
        n106 = Build Array(w279) -> (w280:refnum<vi>[])
        n107 = call "Set Enable State on Multiple Controls.vi"("Enable?"=TRUE, "Controls"=w280) -> ()  [unwired: 10 in]
        n108 = call "Set Enable State on Multiple Controls.vi"("Enable?"=FALSE, "Controls"=w281) -> ()  [unwired: 10 in]
      }
      frame "UI: Update When Stop" {
        # "Enable: Start, Exit, Settings\nDisable: Stop"
        n109 = Unbundle By Name(w286) -> ("UI Refs.Stop Ref"=w291:refnum<vi>, "UI Refs.Start Ref"=w292:refnum<vi>, "UI Refs.Exit Ref"=w293:refnum<vi>, "UI Refs.Settings Ref"=w294:refnum<vi>, "UI Refs.Data Source Ref"=w285:refnum<vi>)
        n110 = Build Array(w292, w293, w294, w285) -> (w289:refnum<vi>[])
        n111 = Build Array(w291) -> (w290:refnum<vi>[])
        n112 = call "Set Enable State on Multiple Controls.vi"("Enable?"=FALSE, "Controls"=w290) -> ()  [unwired: 10 in]
        n113 = call "Set Enable State on Multiple Controls.vi"("Enable?"=TRUE, "Controls"=w289) -> ()  [unwired: 10 in]
      }
      frame "UI: Cursor Set" {
        # "Argument"
        # "Set and Unset Cursor Busy.\n(Usage: \"UI: Cursor Set >> Busy|Idle\")"
        n114 = disable-structure shown="Default" {
          disable-tunnel: w301 -> [w307 w312]
          disable-tunnel: [w306 w312] -> w300
          disable-tunnel: w299 -> [w305 _]
          frame condition #0 (active) {
            n115 = case shown="\"Busy\"" w305 {
              tunnel: w307 -> [w309 w311]
              tunnel: [w308 w310] -> w306
              frame "Idle", Default {
                n116 = call <vilib>:"Unset Busy.vi"("error in (no error)"=w309) -> ("error out"=w308:errorcluster)  [unwired: 10 in]
              }
              frame "Busy" {
                n117 = call <vilib>:"Set Busy.vi"("error in (no error)"=w311) -> ("error out"=w310:errorcluster)  [unwired: 9 in, 1 out]
              }
            }
          }
          frame condition #1 {
          }
        }
        n118 = call <vilib>:"Add State(s) to Queue__JKI_lib_State_Machine.vi"("State(s) in (\"\")"=w304) -> ("States Out"=w303:string)  [unwired: 14 in]
      }
      frame "UI: Front Panel State" {
        # "Argument"
        # "Set Front Panel Open or Closed\n(Usage: \"UI: Front Panel State >> Open|Close\")"
        n119 = Unbundle By Name(w316) -> ("Core.Current VI Reference"=w315:refnum<vi>)
        n120 = case shown="\"Minimize\", \"Minimized\"" w314 {
          tunnel: w318 -> [w326 w341 w352 w365 w378]
          tunnel: [w328 w342 w354 w367 w380] -> w317
          tunnel: w315 -> [w327 w339 w353 w366 w379]
          frame "Open", "Standard", Default {
            w321 = T3."Standard" ("State")
            n121 = property class="VI"(reference=w327, error in=w326) -> (reference out=w324:refnum<vi>, error out=w325:errorcluster, "FP.State"=w323:T3)
            n122 = Not Equal?(x=w323, y=w321) -> (x != y?=w322:bool)
            n123 = case shown="True" w322 {
              tunnel: [w332 w334] -> w328
              tunnel: w325 -> [w331 w334]
              tunnel: w324 -> [w330 _]
              tunnel: w321 -> [w329 _]
              frame True {
                n124 = invoke class="VI" method="FP.Open"(reference=w330, error in=w331, "Activate"=TRUE, "State"=w329) -> (error out=w332:errorcluster)  [unwired: 1 in, 4 out]
              }
              frame False {
              }
            }
          }
          frame "Close", "Closed" {
            n125 = property class="VI"(reference=w339, error in=w341) -> (reference out=w338:refnum<vi>, error out=w340:errorcluster, "FP.State"=w336:T3)
            n126 = Not Equal?(x=w336, y=T3."Closed" ("Front Panel Window:State")) -> (x != y?=w335:bool)
            n127 = case shown="True" w335 {
              tunnel: [w343 w346] -> w342
              tunnel: w340 -> [w343 w345]
              tunnel: w338 -> [_ w344]
              frame False {
              }
              frame True {
                n128 = invoke class="VI" method="FP.Close"(reference=w344, error in=w345) -> (error out=w346:errorcluster)  [unwired: 1 in, 2 out]
              }
            }
          }
          frame "Hidden", "Hide" {
            w347 = T3."Hidden" ("State")
            n129 = property class="VI"(reference=w353, error in=w352) -> (reference out=w350:refnum<vi>, error out=w351:errorcluster, "FP.State"=w349:T3)
            n130 = Not Equal?(x=w349, y=w347) -> (x != y?=w348:bool)
            n131 = case shown="True" w348 {
              tunnel: [w358 w359] -> w354
              tunnel: w351 -> [w357 w359]
              tunnel: w350 -> [w356 _]
              tunnel: w347 -> [w355 _]
              frame True {
                n132 = invoke class="VI" method="FP.Open"(reference=w356, error in=w357, "State"=w355) -> (error out=w358:errorcluster)  [unwired: 2 in, 4 out]
              }
              frame False {
              }
            }
          }
          frame "Minimize", "Minimized" {
            w360 = T3."Minimized" ("State")
            n133 = property class="VI"(reference=w366, error in=w365) -> (reference out=w363:refnum<vi>, error out=w364:errorcluster, "FP.State"=w362:T3)
            n134 = Not Equal?(x=w362, y=w360) -> (x != y?=w361:bool)
            n135 = case shown="True" w361 {
              tunnel: [w371 w372] -> w367
              tunnel: w364 -> [w370 w372]
              tunnel: w363 -> [w369 _]
              tunnel: w360 -> [w368 _]
              frame True {
                n136 = invoke class="VI" method="FP.Open"(reference=w369, error in=w370, "State"=w368) -> (error out=w371:errorcluster)  [unwired: 2 in, 4 out]
              }
              frame False {
              }
            }
          }
          frame "Maximize", "Maximized" {
            w373 = T3."Maximized" ("State")
            n137 = property class="VI"(reference=w379, error in=w378) -> (reference out=w376:refnum<vi>, error out=w377:errorcluster, "FP.State"=w375:T3)
            n138 = Not Equal?(x=w375, y=w373) -> (x != y?=w374:bool)
            n139 = case shown="True" w374 {
              tunnel: [w384 w385] -> w380
              tunnel: w377 -> [w383 w385]
              tunnel: w376 -> [w382 _]
              tunnel: w373 -> [w381 _]
              frame True {
                n140 = invoke class="VI" method="FP.Open"(reference=w382, error in=w383, "State"=w381) -> (error out=w384:errorcluster)  [unwired: 2 in, 4 out]
              }
              frame False {
              }
            }
          }
        }
        n141 = call <vilib>:"Add State(s) to Queue__JKI_lib_State_Machine.vi"("State(s) in (\"\")"=w320) -> ("States Out"=w319:string)  [unwired: 14 in]
      }
      frame "UI: Change Waveform Graph Legend Num" {
        n142 = Unbundle By Name(w392) -> ("UI Refs.Data Ref"=w391:refnum<vi>)
        n143 = call "Convert API String Arguments to Data.vim"("Reference Type"=u32 0 ("Legend:Number of Rows"), "API String"=w389) -> ("error out"=w387:errorcluster, "Data"=w390:u32)  [unwired: 6 in]
        n144 = property class="WFChart (strict)"(reference=w391, error in=w387, "LegNumRows"=w390) -> (error out=w386:errorcluster)  [unwired: 1 out]
      }
      frame "UI: Update Waveform Graph" {
        n145 = call "CSM - Convert Argument to MassData.vim"("Type"=waveform(dbl)[] [] ("Data"), "MassData Argument"=w407) -> ("error out"=w405:errorcluster, "Data"=w401:waveform(dbl)[])  [unwired: 6 in]
        "WaveformGraph" <- w401
        n146 = Array Size(array=w401) -> (size(s)=w398:i32)
        n147 = feedback-in #1(w398) -> ()
        n148 = feedback #1(0) -> (w399:i32)
        n149 = Not Equal?(x=w398, y=w399) -> (x != y?=w395:bool)
        n150 = Format Into String(w398) -> (resulting string=w400:string)  [unwired: 3 in, 1 out]
        n151 = call <vilib>:"Build State String with Arguments__JKI_lib_State_Machine.vi"("Arguments (\"\")"=w400, "State"="UI: Change Waveform Graph Legend Num") -> ("State with Arguments"=w396:string)  [unwired: 4 in]
        n152 = call-poly <userlib>:"Add State(s) to Queue By BOOL++.vi"("TRUE (\"\")"=w396, "Condition"=w395, "State Queue (\"\")"=w403) -> ("Remaining States"=w404:string)  [unwired: 8 in]
      }
      frame "UI: Update AnalysisWnd 1" {
        n153 = call "CSM - Convert Argument to MassData.vim"("Type"=cluster{"f0":dbl, "df":dbl, "magnitude":dbl[]}[] [] ("FFT - (RMS)"), "MassData Argument"=w413) -> ("error out"=w412:errorcluster, "Data"=→"AnalysisWnd 1":cluster{"f0":dbl, "df":dbl, "magnitude":dbl[]}[])  [unwired: 6 in]
      }
      frame "UI: Update AnalysisWnd 2" {
        n154 = call "CSM - Convert Argument to MassData.vim"("Type"=cluster{"f0":dbl, "df":dbl, "magnitude":dbl[]}[] [] ("FFT - (RMS)"), "MassData Argument"=w420) -> ("error out"=w419:errorcluster, "Data"=→"AnalysisWnd 2":cluster{"f0":dbl, "df":dbl, "magnitude":dbl[]}[])  [unwired: 6 in]
      }
      frame "---------- Macro ----------" {
        n155 = call <vilib>:"Add State(s) to Queue__JKI_lib_State_Machine.vi"("State(s) in (\"\")"=w428) -> ("States Out"=w427:string)  [unwired: 14 in]
      }
      frame "Macro: Initialize" {
        w429 = "Data: Initialize\nInitialize Core Data\nEvents: Register\nUI: Initialize\nUI: Front Panel State >> Open\nUI: Change Waveform Graph Legend Num >> 1\nDO: Update Status >> Ready...\n\n//Permanent registrations\nAcquired Waveform@Acquisition >> API: Log@Logging -><register>\nAcquired Waveform@Acquisition >> UI: Update Waveform Graph -><register>\n\n//Dynamic registrations\nMacro: Register Analysis Relationships\n\n//Launch Acquisition Module\nMacro: Launch Acquisition Module"  # Data: Initialize Initialize Core Data Events: Register UI: Initialize UI: Front Panel State >> Open UI: Change Waveform Graph Legend Num >> 1 DO: Update Status >> Ready...  //Permanent registrations Acquired Waveform@Acquisition >> API: Log@Logging -><register> Acquired Waveform@Acquisition >> UI: Update Waveform Graph -><register>  //Dynamic registrations Macro: Register Analysis Relationships  //Launch Acquisition Module Macro: Launch Acquisition Module
        # "Initialization Macro\n(This is called once, when the VI starts)"
        n156 = call <userlib>:"CSM - Populate Configuration Variables.vi"("String with INI-Variable"=w429) -> ("String"=w430:string)  [unwired: 7 in, 1 out]
        n157 = call <vilib>:"Add State(s) to Queue__JKI_lib_State_Machine.vi"("State(s) in Front (\"\")"=w430, "State(s) in (\"\")"=w435) -> ("States Out"=w434:string)  [unwired: 13 in]
      }
      frame "Macro: Launch Acquisition Module" {
        n158 = local read "Data Source"() -> (w438:enum16{"Simulated Waveform", "Sound Card"})
        n159 = case shown="\"Simulated Waveform\", Default" w438 {
          tunnel: ["Do: Launch Simulated Acquisition Module" ("State(s) in (\"\")") "Do: Launch Sound Card Acquisition Module" ("State(s) in (\"\")")] -> w437
          frame "Simulated Waveform", Default {
          }
          frame "Sound Card" {
          }
        }
        n160 = call <vilib>:"Add State(s) to Queue__JKI_lib_State_Machine.vi"("State(s) in (\"\")"="Do: Exit Acquisition Module If Exist" ("State(s) in (\"\")"), "State(s) at Back (\"\")"=w437) -> ("States Out"=w436:string)  [unwired: 13 in]
        n161 = call <vilib>:"Add State(s) to Queue__JKI_lib_State_Machine.vi"("State(s) in Front (\"\")"=w436, "State(s) in (\"\")"=w440) -> ("States Out"=w441:string)  [unwired: 13 in]
      }
      frame "Macro: Register Analysis Relationships" {
        # "<2>"
        # "<1>"
        # "#CSM-NOTE\n<1> and <2> will be replaced."
        # "#CSM-NOTE\nState could be registered as status. It's similar to Status with response as its argument."
        n162 = Format Into String("Analysis Window 1") -> (resulting string=w448:string)  [unwired: 3 in, 1 out]
        n163 = Format Into String("Analysis Window 2") -> (resulting string=w447:string)  [unwired: 3 in, 1 out]
        n164 = call-poly <userlib>:"Build Message with Arguments++.vi"("States With Replace Token"="//Dynamic registrations\n\n//For AnalysisWnd 1\nAcquired Waveform@Acquisition >> API: <1>@Algorithm -><register>\nAPI: <1>@Algorithm >> UI: Update AnalysisWnd 1 -><register>\n//For AnalysisWnd 2\nAcquired Waveform@Acquisition >> API: <2>@Algorithm -><register>\nAPI: <2>@Algorithm >> UI: Update AnalysisWnd 2 -><register>" ("State(s) in Front (\"\")"), "<1>"=w448, "<2>"=w447) -> ("States"=w451:string)  [unwired: 12 in]
        n165 = Bundle By Name(cluster=w457, "Relationships"=w451) -> (w453:T9)
        n166 = call <vilib>:"Add State(s) to Queue__JKI_lib_State_Machine.vi"("State(s) in Front (\"\")"=w451, "State(s) in (\"\")"=w454) -> ("States Out"=w455:string)  [unwired: 13 in]
      }
      frame "Macro: Unregister Analysis Relationships" {
        n167 = Unbundle By Name(w469) -> ("Relationships"=w468:string)
        n168 = Search and Replace String(replace all?=TRUE ("ignore case? (F)"), case sensitive?=TRUE ("ignore case? (F)"), input string=w468, search string="<register>" ("replace string (\"\")"), replace string="<unregister>" ("replace string (\"\")")) -> (result string=w461:string)  [unwired: 3 in, 3 out]
        n169 = Bundle By Name(cluster=w469, "Relationships"="") -> (w460:T9)
        n170 = call <vilib>:"Add State(s) to Queue__JKI_lib_State_Machine.vi"("State(s) in Front (\"\")"=w461, "State(s) in (\"\")"=w462) -> ("States Out"=w463:string)  [unwired: 13 in]
      }
      frame "Macro: Start" {
        n171 = Bundle By Name(cluster=w476, "State"=UI_State."Acquiring and Logging" ("UI State")) -> (w475:T9)
        n172 = call <vilib>:"Add State(s) to Queue__JKI_lib_State_Machine.vi"("State(s) in Front (\"\")"="//Local States\nDO: Update Status >> Acquiring and Logging...\nUI: Update When Start\n\n//Send Message to Other CSM Modules\nAPI: Start -@ Logging\nAPI: Start ->| Acquisition" ("State(s) in Front (\"\")"), "State(s) in (\"\")"=w473) -> ("States Out"=w474:string)  [unwired: 13 in]
      }
      frame "Macro: Stop" {
        n173 = Unbundle By Name(w480) -> ("State"=w482:T5)
        n174 = case shown="Default" w482 {
          selector: w482 -> [w489 _]
          tunnel: [w489 UI_State."Waiting for Stop" ("UI State")] -> w481
          frame "Waiting for Exit" {
          }
          frame Default {
          }
        }
        n175 = Bundle By Name(cluster=w480, "State"=w481) -> (w486:T9)
        n176 = call <vilib>:"Add State(s) to Queue__JKI_lib_State_Machine.vi"("State(s) in Front (\"\")"="//Local States\nDO: Update Status >> Stopping...\nUI: Update When Stop\n\n//Send Message to Other CSM Modules\nAPI: Stop -@ Acquisition\nAPI: Stop -@ Logging\n" ("State(s) in Front (\"\")"), "State(s) in (\"\")"=w484) -> ("States Out"=w485:string)  [unwired: 13 in]
      }
      frame "Macro: Exit" {
        w498 = "//UI: Front Panel State >> Close"  # //UI: Front Panel State >> Close
        w495 = "//Dynamic registrations\nMacro: Unregister Analysis Relationships\n\n//Permanent registrations\nAcquired Waveform@Acquisition >> API: Log@Logging -><unregister>\nAcquired Waveform@Acquisition >> UI: Update Waveform Graph -><unregister>\n\nData: Cleanup\nEvents: Unregister\nExit"  # //Dynamic registrations Macro: Unregister Analysis Relationships  //Permanent registrations Acquired Waveform@Acquisition >> API: Log@Logging -><unregister> Acquired Waveform@Acquisition >> UI: Update Waveform Graph -><unregister>  Data: Cleanup Events: Unregister Exit
        # "Exit Macro\n(This is called once, when the VI exits)"
        n177 = Unbundle By Name(w500) -> ("Core.Close Panel on Exit?"=w499:bool)
        n178 = disable-structure shown="Enabled" {
          disable-tunnel: [w503 w515 w521] -> w492
          disable-tunnel: w491 -> [_ w514 _]
          frame Disabled {
            w510 = "Macro: Exit -@ Acquisition\nMacro: Exit -@ Logging"  # Macro: Exit -@ Acquisition Macro: Exit -@ Logging
            n179 = call <userlib>:"CSM - Module Status.vi"("CSM Name"="Algorithm") -> ("#Nodes"=w506:i32, "CSM Name (Dup)"=w508:string)  [unwired: 6 in, 3 out]
            n180 = for {
              N: w506 -> [_]
              tunnel: w508 -> [w513]
              tunnel: "Macro: Exit" -> [w512]
              tunnel: [w511] -> w504 mode=indexing
              n181 = call-poly <userlib>:"Build Message with Arguments++.vi"("State With Arguments"=w512, "Target Module (\"\")"=w513) -> ("CSM Message String"=w511:string)  [unwired: 13 in]
            }
            n182 = Build Array (concatenate)(w510, w504) -> (w505:string[])
            n183 = call <userlib>:"CSM - Compact Multiple States.vi"("Multiple States"=w505) -> ("States"=w503:string)  [unwired: 9 in]
          }
          frame Enabled {
            # "#NOTE\nHelper VI is equivalent to other case"
            n184 = call <userlib>:"CSM - List Modules.vi"() -> ("Module Names"=w517:string[])  [unwired: 10 in, 1 out]
            n185 = Search 1D Array(1D array=w517, element=w514) -> (index of element=w518:i32)  [unwired: 1 in]
            n186 = Delete From Array(array=w517, index=w518) -> (array with subset deleted=w516:string[])  [unwired: 1 in, 1 out]
            n187 = call <userlib>:"CSM - Build Exit Messages of CSMs.vi"("State With Arguments (\"Macro: Exit“)"="Macro: Exit" ("State with Arguments(\"Macro: Exit“)"), "CSMs"=w516) -> ("States"=w515:string)  [unwired: 13 in]
          }
          frame Disabled {
            # "#NOTE\nHelper VI is equivalent to other case"
            n188 = call <userlib>:"CSM - Build Exit Messages of CSMs.vi"("State With Arguments (\"Macro: Exit“)"="Macro: Exit" ("State with Arguments(\"Macro: Exit“)"), "CSMs"=string[] ["Acquisition", "Logging", "Algorithm"]) -> ("States"=w521:string)  [unwired: 13 in]
          }
        }
        n189 = Select(t=w498, s=w499, f="") -> (s? t:f=w496:string)
        n190 = call <vilib>:"Add State(s) to Queue__JKI_lib_State_Machine.vi"("State(s) in Front (\"\")"=w492, "State(s) in (\"\")"=w496, "State(s) at Back (\"\")"=w495) -> ("States Out"=w494:string)  [unwired: 12 in]
        n191 = call <vilib>:"Add State(s) to Queue__JKI_lib_State_Machine.vi"("State(s) in Front (\"\")"=w494, "State(s) in (\"\")"=w502) -> ("States Out"=w501:string)  [unwired: 13 in]
      }
      frame "---------- DoSth ----------" {
        n192 = call <vilib>:"Add State(s) to Queue__JKI_lib_State_Machine.vi"("State(s) in (\"\")"=w527) -> ("States Out"=w526:string)  [unwired: 14 in]
      }
      frame "Do: Update Status" {
        n193 = call <vilib>:"Add State(s) to Queue__JKI_lib_State_Machine.vi"("State(s) in (\"\")"=w533) -> ("States Out"=w532:string)  [unwired: 14 in]
        "Status" <- w528
      }
      frame "Do: Launch Settings Dialog" {
        # "Your code here.\n(You can make a copy of, or modify, this frame)"
        n194 = call <userlib>:"CSM - Check If Module Exists.vi"("CSM Name"="Acquisition" ("Name(\"\" to use uuid)")) -> ("error out"=w540:errorcluster, "Exist?"=w536:bool, "CSM Name (Dup)"=w538:string)  [unwired: 8 in]
        n195 = case shown="True" w536 {
          tunnel: w540 -> [w548 w560]
          tunnel: w538 -> [w544 w559]
          tunnel: w537 -> [_ w558]
          tunnel: [w547 w557] -> w535
          frame False {
            n196 = Format Into String(format string="Cannot Find the CSM which named %s !!!", w544) -> (resulting string=w543:string)  [unwired: 2 in, 1 out]
            n197 = Bundle By Name(cluster=w548, "status"=TRUE, "source"=w543) -> (w547:errorcluster)
          }
          frame True {
            w552 = T3."Standard" ("State")
            n198 = call <userlib>:"CSM - Module VI Reference.vi"("Current Module (\"\" to Generate an ID)"=w558, "error in (no error)"=w560, "Force? (F)"=TRUE ("force?(F)"), "CSM Name"=w559) -> ("error out"=w550:errorcluster, "CSM Module VIRef"=w551:refnum<vi>)  [unwired: 6 in]
            n199 = property class="VI"(reference=w551, error in=w550) -> (reference out=w555:refnum<vi>, error out=w556:errorcluster, "FP.State"=w554:T3)
            n200 = Not Equal?(x=w554, y=w552) -> (x != y?=w553:bool)
            n201 = case shown="True" w553 {
              tunnel: [w567 w569] -> w557
              tunnel: w556 -> [w562 w569]
              tunnel: w555 -> [w561 _]
              tunnel: w552 -> [w566 _]
              frame True {
                n202 = property class="VI"(reference=w561, error in=w562, "FP.Behavior"=T6."Modal" ("Front Panel Window:Behavior")) -> (reference out=w564:refnum<vi>, error out=w565:errorcluster)
                n203 = invoke class="VI" method="FP.Open"(reference=w564, error in=w565, "Activate"=TRUE, "State"=w566) -> (error out=w567:errorcluster)  [unwired: 1 in, 4 out]
              }
              frame False {
              }
            }
          }
        }
      }
      frame "Do: Confirm Quit" {
        n204 = Unbundle By Name(w574) -> ("State"=w577:T5)
        n205 = case shown="\"Acquiring and Logging\"" w577 {
          tunnel: [UI_State."Idle" ("UI State") w586] -> w576
          tunnel: w574 -> [w581 w585]
          tunnel: [w581 w584] -> w575
          tunnel: [TRUE w583] -> w570
          frame Default {
          }
          frame "Acquiring and Logging" {
            n206 = Two Button Dialog(message="Are you sure you want to quit while the acquisition is running?" ("Confirm Quit Message"), 1:"No" ("No"), 2:"Yes" ("Yes")) -> (T button?=w587:bool)
            n207 = case shown="False" w587 {
              tunnel: [UI_State."Acquiring and Logging" ("UI State") UI_State."Waiting for Exit" ("UI State")] -> w586
              tunnel: w585 -> [w591 w594]
              tunnel: [w591 w594] -> w584
              tunnel: [_ TRUE] -> w583
              frame False {
                # "User did not want to quit."
              }
              frame True {
              }
            }
          }
        }
        n208 = Bundle By Name(cluster=w575, "State"=w576) -> (w573:T9)
        n209 = call-poly <userlib>:"Add State(s) to Queue By BOOL++.vi"("TRUE (\"\")"="Macro: Exit", "Condition"=w570, "State Queue (\"\")"=w579) -> ("Remaining States"=w572:string)  [unwired: 8 in]
      }
      frame "Do: Exit Acquisition Module If Exist" {
        n210 = call <userlib>:"CSM - Check If Module Exists.vi"("CSM Name"="Acquisition") -> ("error out"=w600:errorcluster, "Exist?"=w597:bool, "CSM Name (Dup)"=w598:string)  [unwired: 8 in]
        n211 = case shown="True" w597 {
          tunnel: w600 -> [w605 w610]
          tunnel: w599 -> [_ w609]
          tunnel: w598 -> [_ w607]
          tunnel: [w605 w606] -> w596
          frame False {
          }
          frame True {
            n212 = call <userlib>:"CSM - Send Message and Wait for Reply.vi"("Current Module (\"\" to Generate an ID)"=w609, "Error In (No Error)"=w610, "Target Module"=w607, "State"="Macro: Exit") -> ("error out"=w606:errorcluster)  [unwired: 5 in, 2 out]
          }
        }
      }
      frame "Do: Launch Simulated Acquisition Module" {
        w611 = "Acquisition"  # Name("" to use uuid)
        n213 = vi-ref "Acquisition.lvlib:Acquisition.vi"() -> (w615:refnum<vi>)
        n214 = property class="VI Interface Type 2"(reference=w615) -> (reference out=w619:refnum<vi>, error out=w617:errorcluster, "Path"=w616:path)  [unwired: 1 in]
        n215 = Open VI Reference(type specifier VI Refnum (for type only)=w619, vi path=w616, options=128, error in (no error)=w617) -> (vi reference=w618:refnum<vi>, error out=w614:errorcluster)  [unwired: 2 in]
        n216 = call-by-ref "Start Asynchronous Call"(reference=w618, error in=w614, "Name(\"\" to use uuid)"=w611) -> (reference out=w621:refnum<vi>, error out=w620:errorcluster)  [unwired: 11 in]
        n217 = Close Reference(reference=w621, error in (no error)=w620) -> (error out=w613:errorcluster)
        n218 = call <userlib>:"CSM - Wait for Module to Be Alive.vi"("CSM Name"=w611, "error in (no error)"=w613) -> ("error out"=w612:errorcluster)  [unwired: 11 in, 2 out]
      }
      frame "Do: Launch Sound Card Acquisition Module" {
        w626 = "Acquisition"  # Name("" to use uuid)
        n219 = vi-ref "SoundInput-DAQ.lvlib:SoundInput-DAQ.vi"() -> (w630:refnum<vi>)
        n220 = property class="VI Interface Type 2"(reference=w630) -> (reference out=w634:refnum<vi>, error out=w632:errorcluster, "Path"=w631:path)  [unwired: 1 in]
        n221 = Open VI Reference(type specifier VI Refnum (for type only)=w634, vi path=w631, options=128, error in (no error)=w632) -> (vi reference=w633:refnum<vi>, error out=w629:errorcluster)  [unwired: 2 in]
        n222 = call-by-ref "Start Asynchronous Call"(reference=w633, error in=w629, "Name(\"\" to use uuid)"=w626) -> (reference out=w636:refnum<vi>, error out=w635:errorcluster)  [unwired: 11 in]
        n223 = Close Reference(reference=w636, error in (no error)=w635) -> (error out=w628:errorcluster)
        n224 = call <userlib>:"CSM - Wait for Module to Be Alive.vi"("CSM Name"=w626, "error in (no error)"=w628) -> ("error out"=w627:errorcluster)  [unwired: 11 in, 2 out]
      }
    }
  }
  n225 = call <userlib>:"CSM - Sync Configuration Variables to File.vi"("All Temp Variable to Default Ini(F)"=TRUE, "error in (no error)"=w2) -> ("error out"=w1:errorcluster)  [unwired: 7 in]
  n226 = disable-structure shown="RUN_TIME_ENGINE==True" {
    disable-tunnel: w1 -> [_ _]
    frame condition #0 (active) {
    }
    frame condition #1 {
      n227 = Quit LabVIEW(quit? (T)=TRUE) -> ()
    }
  }
